vi "Initialize Network.vi"(8 "error in (no error)":errorcluster, 11 "Settings  in":T1={"UDP Receiver"=refnum, "UDP Sender"=refnum, "Valid Packet"=FALSE, "TCP"=refnum, "Network Settings"={"IP adress"="127.0.0.1", "RDB"={"Protocol"=enum."UDP", "Tx Port"=48270, "Rx Port"=10, "Buffer Size"=204800, "Timeout"=10}, "SCP"={"Protocol"=enum."TCP", "Tx Port"=48191, "Rx Port"=48191, "Buffer Size"=204800, "Timeout"=10}}, "vclient"=path "", "paeseHandle"=0, "builderHandle"=0}) -> (0 "error out":errorcluster, 3 "Settings out":T1={"UDP Receiver"=refnum, "UDP Sender"=refnum, "Valid Packet"=FALSE, "TCP"=refnum, "Network Settings"={"IP adress"="127.0.0.1", "RDB"={"Protocol"=enum."UDP", "Tx Port"=48270, "Rx Port"=10, "Buffer Size"=204800, "Timeout"=10}, "SCP"={"Protocol"=enum."TCP", "Tx Port"=48191, "Rx Port"=48191, "Buffer Size"=204800, "Timeout"=10}}, "vclient"=path "", "paeseHandle"=0, "builderHandle"=0})   [LabVIEW 2023, in "Vires VTD Engine.lvlib"]
uses:
  Vires VTD Engine.lvlib
  Type/Settings.ctl
  Shared/Network Settings.ctl
  Shared/Protocol.ctl
  Shared/Vires VTD Shared.lvlib
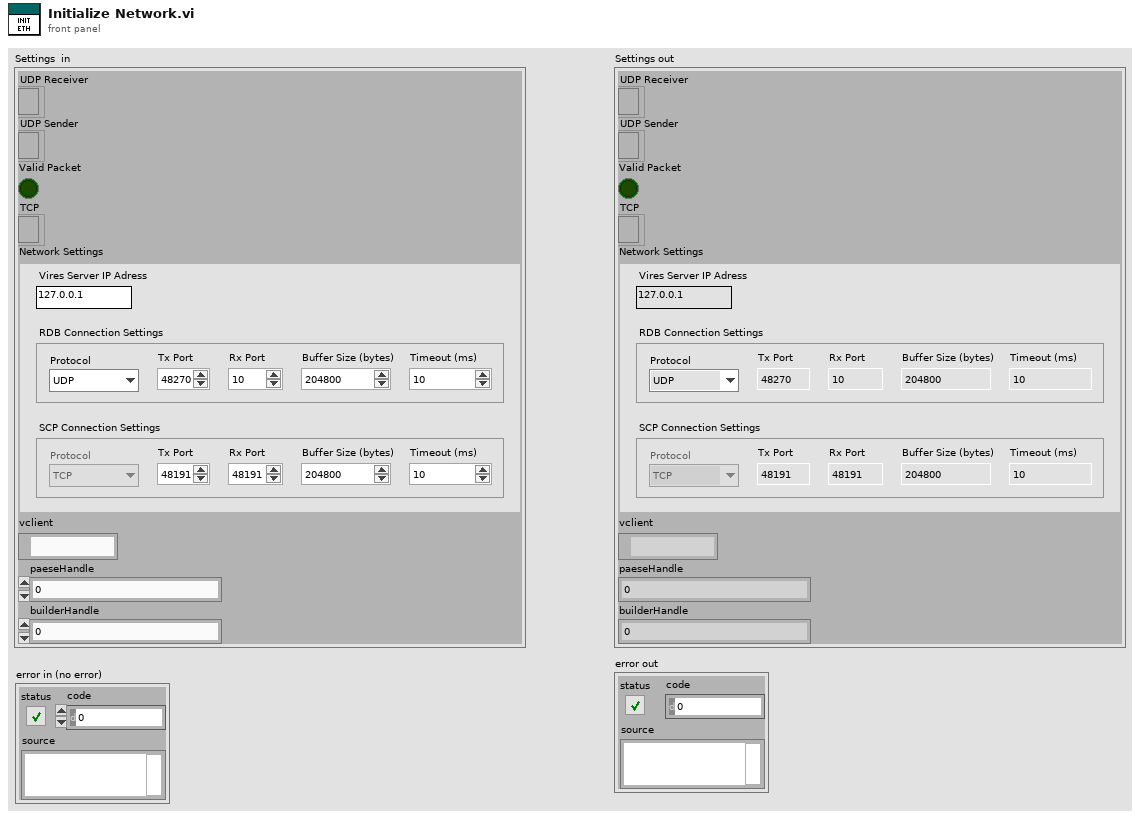
[diagram p1: front panel]
types:
  T1 = typedef "Vires VTD Engine.lvlib/Settings.ctl" = cluster{"UDP Receiver":refnum<k16>, "UDP Sender":refnum<k16>, "Valid Packet":bool, "TCP":refnum<k5>, "Network Settings":T2, "vclient":path, "paeseHandle":u64, "builderHandle":u64}
  T2 = typedef "Vires VTD Shared.lvlib/Network Settings.ctl" = cluster{"IP adress":string, "RDB":cluster{"Protocol":T3, "Tx Port":u16, "Rx Port":u16, "Buffer Size":i32, "Timeout":u16}, "SCP":cluster{"Protocol":T3, "Tx Port":u16, "Rx Port":u16, "Buffer Size":i32, "Timeout":u16}}
  T3 = typedef "Vires VTD Shared.lvlib/Protocol.ctl" = enum16{"UDP", "TCP"}
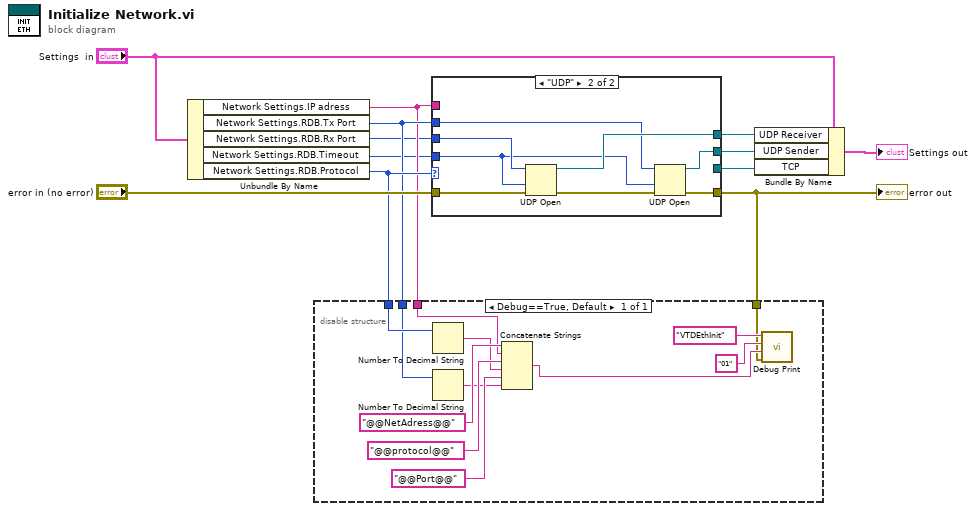
[diagram p0: block diagram]
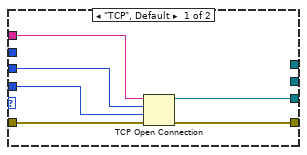
[diagram p2: hidden frame]
diagram:
  n1 = Unbundle By Name("Settings  in") -> ("Network Settings.IP adress"=w4:string, "Network Settings.RDB.Tx Port"=w5:u16, "Network Settings.RDB.Rx Port"=w2:u16, "Network Settings.RDB.Timeout"=w1:u16, "Network Settings.RDB.Protocol"=w6:T3)
  n2 = case shown="\"UDP\"" w6 {
    tunnel: "error in (no error)" -> [w18 w26]
    tunnel: [w17 w24] -> w7
    tunnel: [_ w23] -> w11
    tunnel: [w16 _] -> w9
    tunnel: [_ w22] -> w8
    tunnel: w4 -> [w15 _]
    tunnel: w5 -> [_ w21]
    tunnel: w2 -> [w13 w20]
    tunnel: w1 -> [w14 w19]
    frame "TCP", Default {
      n3 = TCP Open Connection(address=w15, remote port or service name=w13, timeout ms (60000)=w14, error in (no error)=w18) -> (connection ID=w16:refnum<k5>, error out=w17:errorcluster)  [unwired: 1 in]
    }
    frame "UDP" {
      n4 = UDP Open(8:w26, 9:w19, 11:w20) -> (port=w22:refnum<k16>, 0:w25:errorcluster)  [unwired: 2 in, 1 out]
      n5 = UDP Open(8:w25, 9:w19, 11:w21) -> (port=w23:refnum<k16>, 0:w24:errorcluster)  [unwired: 2 in, 1 out]
    }
  }
  "error out" <- w7
  n6 = disable-structure shown="Debug==True, Default" {
    disable-tunnel: w5 -> [w27]
    disable-tunnel: w6 -> [w28]
    disable-tunnel: w4 -> [w30]
    disable-tunnel: w7 -> [w29]
    frame condition #0 (active) {
      n7 = Number To Decimal String(number=w28) -> (decimal integer string=w35:string)  [unwired: 1 in]
      n8 = Number To Decimal String(number=w27) -> (decimal integer string=w33:string)  [unwired: 1 in]
      n9 = Concatenate Strings("@@NetAdress@@" ("string"), w30, "@@protocol@@" ("string"), w35, "@@Port@@" ("string"), w33) -> (w32:string)
      n10 = call "Debug Print.vi"("error out"=w29, "comment"=w32, "Index"="01", "Module"="VTDEthInit") -> ()  [unwired: 8 in]
    }
  }
  n11 = Bundle By Name(cluster="Settings  in", "UDP Receiver"=w8, "UDP Sender"=w11, "TCP"=w9) -> (→"Settings out":T1)
